vi "Export.vi"(8 "error in (no error)":errorcluster, 11 "BluelinesRedlines in":refnum<class "BluelinesRedlines.lvclass">) -> (0 "error out":errorcluster, 3 "BluelinesRedlines out":refnum<class "BluelinesRedlines.lvclass">)   [LabVIEW 2020, in "VolatusGUIElements.lvlib" / "BluelinesRedlines.lvclass"]
uses:
  BluelinesRedlines.lvclass
  <vilib>/Utility/sysdir.llb/System Directory Type.ctl
  BluelinesRedlines.lvclass/BluelinesRedlines.ctl
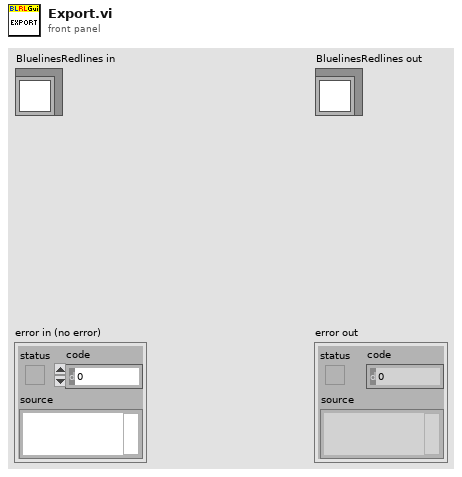
[diagram p1: front panel]
types:
  T1 = typedef "System Directory Type.ctl" = i32
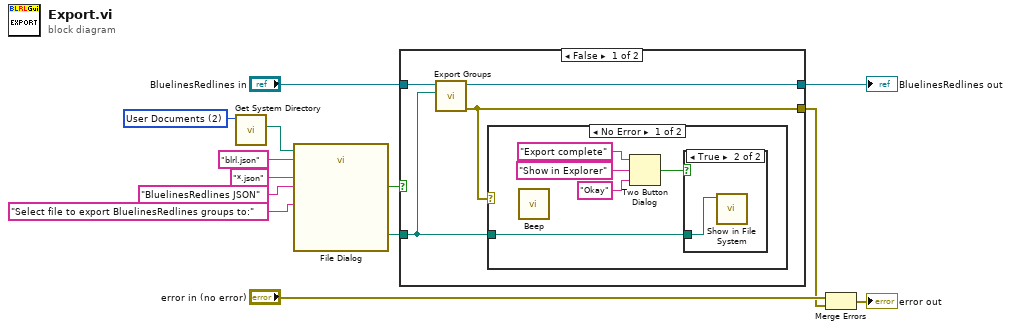
[diagram p0: block diagram]
diagram:
  w12 = T1 2 items=["User Home"=0, "User Desktop"=1, "User Documents"=2, "User Application Data"=3, "User Preferences"=4, "User Temporary"=5, "Public Documents"=6, "Public Application Data"=7, "Public Preferences"=8, "Public Cache"=13, "System Core Libraries"=9, "System Installed Libraries"=10, "Application Files"=11, "Boot Volume Root"=12] ("system directory type")
  n1 = call <vilib>:"Get System Directory.vi"("system directory type"=w12) -> ("system directory"=w11:path)  [unwired: 10 in]
  n2 = call "File Dialog"("start path"=w11, "prompt"="Select file to export BluelinesRedlines groups to:", "default name"="blrl.json", "pattern (all files)"="*.json", "pattern label"="BluelinesRedlines JSON") -> ("selected path"=w5:path, "cancelled"=w6:bool)  [unwired: 7 in, 2 out]
  n3 = case shown="False" w6 {
    tunnel: w5 -> [w14 _]
    tunnel: "BluelinesRedlines in" -> [w17 w24]
    tunnel: [w16 w24] -> w3
    tunnel: [w15 _] -> w1
    frame False {
      n4 = call "Export Groups.vi"("Path"=w14, "BluelinesRedlines in"=w17) -> ("error out"=w15:errorcluster, "BluelinesRedlines out"=w16:refnum<class "BluelinesRedlines.lvclass">)  [unwired: 8 in]
      n5 = case shown="No Error" w15 {
        tunnel: w14 -> [w18 _]
        frame No Error {
          n6 = call <vilib>:"Beep.vi"() -> ()  [unwired: 12 in]
          n7 = Two Button Dialog(message="Export complete", 1:"Okay" ("F button name (\"Cancel\")"), 2:"Show in Explorer" ("T button name (\"OK\")")) -> (T button?=w19:bool)
          n8 = case shown="True" w19 {
            tunnel: w18 -> [_ w23]
            frame False {
            }
            frame True {
              n9 = call <vilib>:"Show in File System.vi"("file or directory path"=w23) -> ()  [unwired: 10 in, 1 out]
            }
          }
        }
        frame Error {
        }
      }
    }
    frame True {
    }
  }
  "BluelinesRedlines out" <- w3
  n10 = Merge Errors("error in (no error)", w1) -> (→"error out":errorcluster)
